vi "Set_Ramps.vi"(8 "error in (no error)":errorcluster, 9 "Decel (ms/krpm)":u16, 10 "Accel (ms/krpm)":u16, 11 "Motor in":refnum<class "Motor.lvclass">) -> (0 "error out":errorcluster, 3 "Motor out":refnum<class "Motor.lvclass">)   [LabVIEW 2021, in "Motor.lvclass"]
uses:
  Motor.lvclass
  Motor.lvclass/Motor.ctl
  ServoDrive/ServoDrive.lvclass
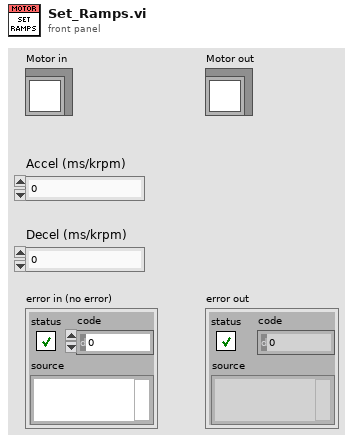
[diagram p1: front panel]
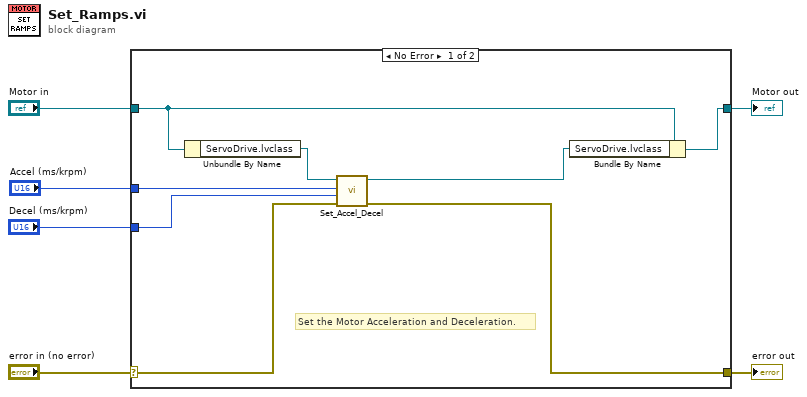
[diagram p0: block diagram]
diagram:
  n1 = case shown="No Error" "error in (no error)" {
    selector: "error in (no error)" -> [w9 w16]
    tunnel: [w8 w16] -> w5
    tunnel: [w12 w15] -> w3
    tunnel: "Motor in" -> [w13 w15]
    tunnel: "Accel (ms/krpm)" -> [w11 _]
    tunnel: "Decel (ms/krpm)" -> [w10 _]
    frame No Error {
      # "Set the Motor Acceleration and Deceleration."
      n2 = Unbundle By Name(w13) -> ("ServoDrive.lvclass"=w14:refnum<class "ServoDrive.lvclass">)
      n3 = call-dynamic "Set_Accel_Decel.vi"("error in (no error)"=w9, "Decel (ms/krpm)"=w10, "Accel (ms/krpm)"=w11, "ServoDrive in"=w14) -> ("error out"=w8:errorcluster, "ServoDrive out"=w7:refnum<class "ServoDrive.lvclass">)  [unwired: 6 in]
      n4 = Bundle By Name(cluster=w13, "ServoDrive.lvclass"=w7) -> (w12:refnum<class "Motor.lvclass">)
    }
    frame Error {
    }
  }
  "error out" <- w5
  "Motor out" <- w3
